vi "SA set Frequency.vi"(8 "error in (no error)":errorcluster caption="에러 입력(에러 없음)", 9 "Stop":dbl, 10 "Start":dbl, 11 "Instrument Manager 입력":refnum<class "Instrument Manager.lvclass">) -> (0 "error out":errorcluster caption="에러 출력", 3 "Instrument Manager 출력":refnum<class "Instrument Manager.lvclass">)   [LabVIEW 2023, in "Instrument Manager.lvclass"]
uses:
  Instrument Manager.lvclass
  Module/Spectrum Analyzer/TYPE DEFINITION/TYPE Start and Stop Frequency.ctl
  Instrument Manager.lvclass/Instrument Manager.ctl
  Module/Spectrum Analyzer/Interface_Spectrum/Interface_Spectrum.lvclass
  Module/Spectrum Analyzer/Spectrum Analyzer.lvlib
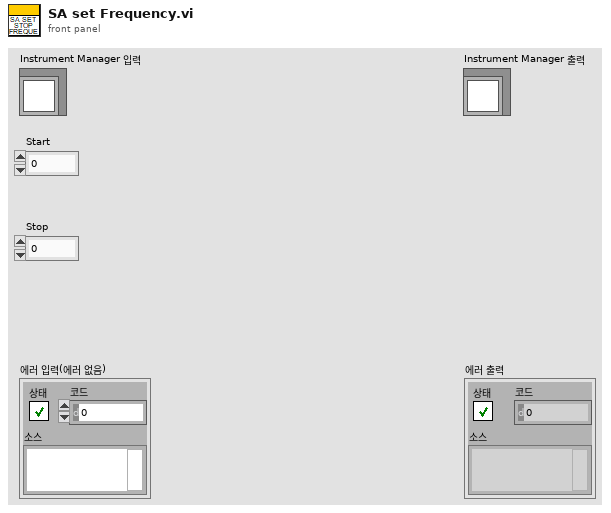
[diagram p1: front panel]
types:
  T1 = typedef "Spectrum Analyzer.lvlib/TYPE Start and Stop Frequency.ctl" = cluster{"Start":dbl, "Stop":dbl}
  T2 = cluster{"Anritsu Call Box":refnum<class "Anritsu Call Box.lvclass">, "Spectrum Analyzer":refnum<class "Interface_Spectrum.lvclass">, "RF Switch Box":refnum<class "RF Filter Box.lvclass">, "Turn Table":refnum<class "Interface - Turn Table.lvclass">, "Mast":refnum<class "Interface - Mast.lvclass">, "3D Controller":refnum<class "Interface_3D Controller.lvclass">}
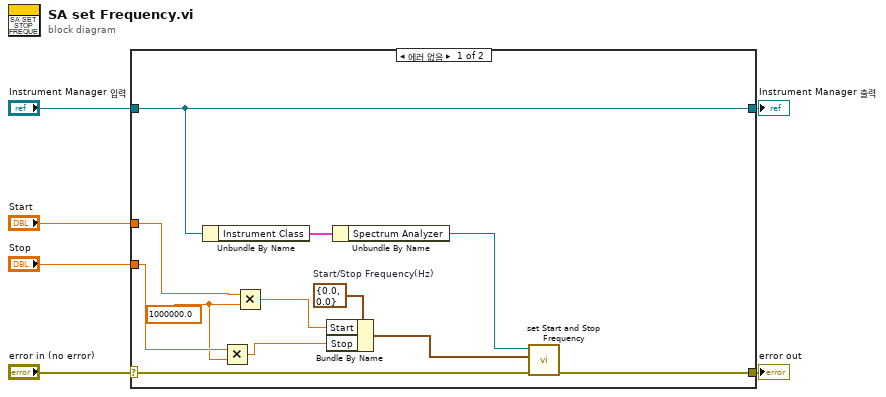
[diagram p0: block diagram]
diagram:
  n1 = case shown="에러 없음" "error in (no error)" {
    selector: "error in (no error)" -> [w15 w20]
    tunnel: [w14 w20] -> w5
    tunnel: [w17 w19] -> w3
    tunnel: "Instrument Manager 입력" -> [w17 w19]
    tunnel: "Start" -> [w11 _]
    tunnel: "Stop" -> [w8 _]
    frame No Error {
      w7 = 1000000.0 ("y")
      w16 = T1 {"Start"=0.0, "Stop"=0.0}  # Start/Stop Frequency(Hz)
      n2 = Unbundle By Name(w17) -> ("Instrument Class"=w18:T2)
      n3 = Multiply(x=w8, y=w7) -> (x*y=w9:dbl)
      n4 = Multiply(x=w11, y=w7) -> (x*y=w10:dbl)
      n5 = Bundle By Name(cluster=w16, "Start"=w10, "Stop"=w9) -> (w12:T1)
      n6 = Unbundle By Name(w18) -> ("Spectrum Analyzer"=w13:refnum<class "Interface_Spectrum.lvclass">)
      n7 = call-dynamic "set Start and Stop Frequency.vi"("error in (no error)"=w15, "Start/Stop Frequency(Hz)"=w12, "Interface_Spectrum in"=w13) -> ("error out"=w14:errorcluster)  [unwired: 7 in, 1 out]
    }
    frame Error {
    }
  }
  "error out" <- w5
  "Instrument Manager 출력" <- w3
